vi "Echo_Classify_API.vi"(8 "error in (no error)":errorcluster, 9 "i":i32, 10 "context":T3 {"ack hi" format="%.0x"; "ack lo" format="%.0x"; "test hi" format="%.0x"; "test lo" format="%.0x"}, 11 "frames":T4 {"flags" format="%.0x"; "id" format="%.0x"}) -> (0 "error out":errorcluster, 3 "frame":T1 {"id" format="%.0x"})   [LabVIEW 2021]
doc: "S5 echo via API: classifies frame i of a CANsub_Frames buffer (from Read): Test / Ack / Other, seq, idx, key, index. Same logic as Echo_Classify. Loop-safe: no allocation, bounded time."
uses:
  Echo_Frame_Kind.ctl
  Echo_Frame.ctl
  Echo_Context.ctl
  api/Typedefs/CANsub_Frames.ctl
  api/CANsub_API.lvlib
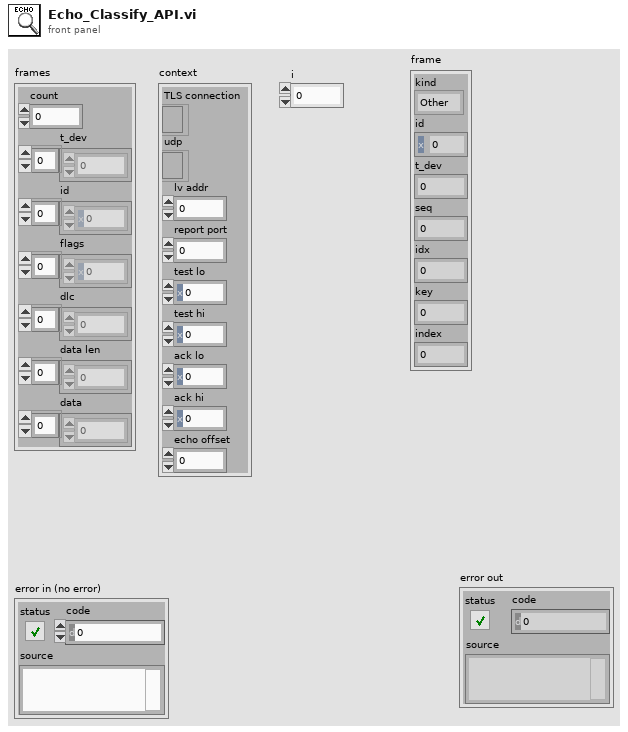
[diagram p1: front panel]
types:
  T1 = typedef "Echo_Frame.ctl" = cluster{"kind":T2, "id":u32, "t_dev":dbl, "seq":u16, "idx":u8, "key":i32, "index":i32}
  T2 = typedef "Echo_Frame_Kind.ctl" = enum16{"Other", "Test", "Ack"}
  T3 = typedef "Echo_Context.ctl" = cluster{"TLS connection":refnum<k5>, "udp":refnum<k16>, "lv addr":u32, "report port":u16, "test lo":u32, "test hi":u32, "ack lo":u32, "ack hi":u32, "echo offset":i32}
  T4 = typedef "CANsub_API.lvlib/CANsub_Frames.ctl" = cluster{"count":i32, "t_dev":dbl[], "id":u32[], "flags":u16[], "dlc":u8[], "data len":u8[], "data":u8[]}
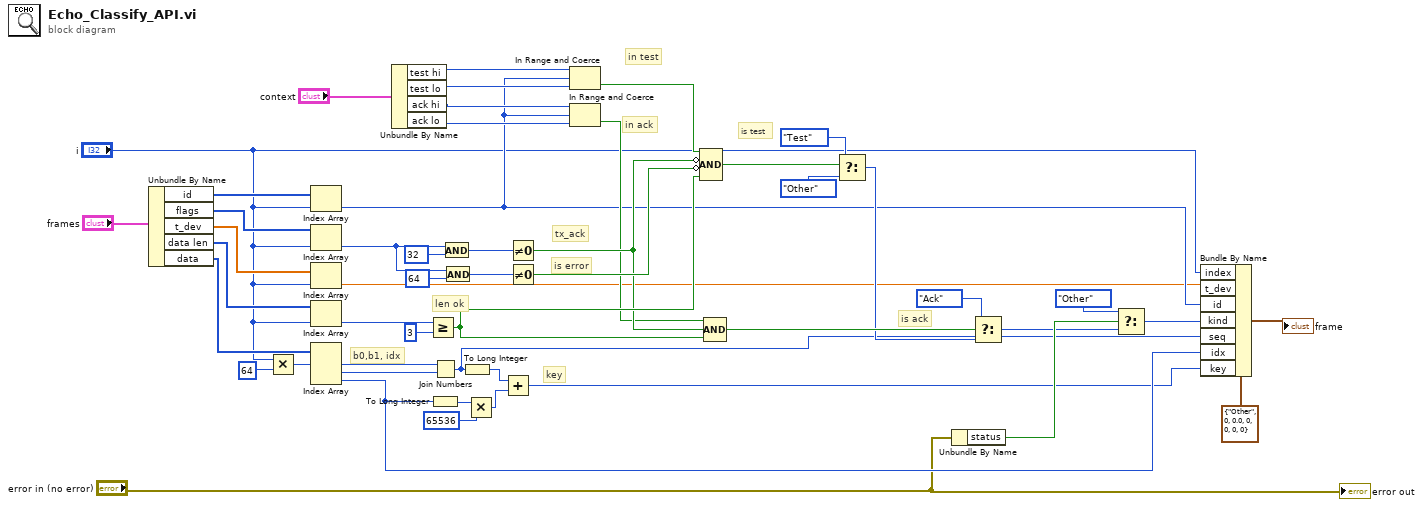
[diagram p0: block diagram]
diagram:
  # "is ack"
  # "is test"
  # "in ack"
  # "in test"
  # "len ok"
  # "key"
  # "b0,b1, idx"
  # "is error"
  # "tx_ack"
  n1 = Unbundle By Name("frames") -> ("id"=w48:u32[], "flags"=w47:u16[], "t_dev"=w46:dbl[], "data len"=w45:u8[], "data"=w38:u8[])
  n2 = Multiply(x="i", y=64) -> (x*y=w37:i32)
  n3 = Index Array(array=w48, index="i") -> (element=w8:u32)
  n4 = Index Array(array=w47, index="i") -> (element=w44:u16)
  n5 = Index Array(array=w46, index="i") -> (element=w7:dbl)
  n6 = Index Array(array=w45, index="i") -> (element=w26:u8)
  n7 = Index Array(array=w38, index #1=w37) -> (element #1=w36:u8, element #2=w35:u8, element #3=w5:u8)  [unwired: 2 in]
  n8 = Unbundle By Name("context") -> ("test hi"=w30:u32, "test lo"=w29:u32, "ack hi"=w28:u32, "ack lo"=w27:u32)
  n9 = Greater Or Equal?(x=w26, y=u8 3) -> (x >= y?=w22:bool)
  n10 = To Long Integer(number=w5) -> (32bit integer=w34:i32)
  n11 = Join Numbers(hi=w36, lo=w35) -> ((hi.lo)=w6:u16)
  n12 = And(x=w44, y=u16 32) -> (x .and. y?=w41:u16)
  n13 = And(x=w44, y=u16 64) -> (x .and. y?=w40:u16)
  n14 = To Long Integer(number=w6) -> (32bit integer=w32:i32)
  n15 = Multiply(x=w34, y=65536) -> (x*y=w31:i32)
  n16 = Add(x=w32, y=w31) -> (x+y=w4:i32)
  n17 = Not Equal To 0?(x=w41) -> (x != 0?=w21:bool)
  n18 = Not Equal To 0?(x=w40) -> (x != 0?=w24:bool)
  n19 = In Range and Coerce(upper limit=w30, x=w8, lower limit=w29) -> (In Range?=w23:bool)  [unwired: 1 out]
  n20 = In Range and Coerce(upper limit=w28, x=w8, lower limit=w27) -> (In Range?=w20:bool)  [unwired: 1 out]
  n21 = Compound Arithmetic op=AND(w23, invert w21, invert w24, w22) -> (w19:bool)
  n22 = Compound Arithmetic op=AND(w20, w21, w22) -> (w18:bool)
  n23 = Select(t=Echo_Frame_Kind."Test" ("Echo_Frame_Kind"), s=w19, f=Echo_Frame_Kind."Other" ("Echo_Frame_Kind")) -> (s? t:f=w14:T2)
  n24 = Unbundle By Name("error in (no error)") -> ("status"=w13:bool)
  n25 = Select(t=Echo_Frame_Kind."Ack" ("Echo_Frame_Kind"), s=w18, f=w14) -> (s? t:f=w12:T2)
  n26 = Select(t=Echo_Frame_Kind."Other" ("Echo_Frame_Kind"), s=w13, f=w12) -> (s? t:f=w9:T2)
  n27 = Bundle By Name(cluster=T1 {"kind"=enum."Other", "id"=0, "t_dev"=0.0, "seq"=0, "idx"=0, "key"=0, "index"=0} ("Echo_Frame"), "index"="i", "t_dev"=w7, "id"=w8, "kind"=w9, "seq"=w6, "idx"=w5, "key"=w4) -> (→"frame":T1)
  "error out" <- "error in (no error)"
